vi "AO.Range to String.vi"(11 "AO.Range":T1) -> (3 "string":string)   [LabVIEW 2019, in "Instrument.Lockin.lvlib" / "Instrument.Lockin.lvclass"]
uses:
  Instrument.Lockin.lvclass
  Lockin.Typedefs/DAQ/DAQ.Config.AO.Range--enum.ctl
  Lockin.Typedefs/Lockin.Typedefs.lvlib
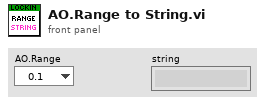
[diagram p1: front panel]
types:
  T1 = typedef "Lockin.Typedefs.lvlib/DAQ.Config.AO.Range--enum.ctl" = enum16{"0.1", "1.0", "3.5", "10.0", ""}
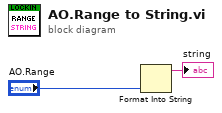
[diagram p0: block diagram]
diagram:
  n1 = Format Into String("AO.Range") -> (resulting string=→"string":string)  [unwired: 3 in, 1 out]
